vi "RemoteVI Menu Click.vi"(0 "hWnd":u64, 1 "button down?":bool, 5 "menus":T1(array[cluster]), 7 "k":i32, 9 "point":cluster{"x":i32, "y":i32}, 11 "error in":errorcluster) -> (4 "handled?":bool, 15 "error out":errorcluster)   [LabVIEW 2020, in "RemoteVI.lvlib"]
doc: "A remote click on an open LabVIEW menu window menus[k] (RemoteVI List Menus.vi, deepest first), done with keys only - no cursor and no window is moved, so every menu stays where LabVIEW put it. A BUTTON-DOWN: on a parent menu (k > 0) on the item that opened the open submenu nothing happens (as locally); otherwise the k submenus above are closed with VK_LEFT (RemoteVI Close Submenus.vi), the highlight is moved onto the clicked item (RemoteVI Highlight Menu Row.vi, VK_DOWN / VK_UP) and, when the item is under the click, VK_RETURN is posted - it chooses the item, or opens its submenu next to the menu when it has one (measured on LabVIEW 2025: plot legend, ring and shortcut menus). A click on a separator or a disabled item moves the highlight but chooses nothing. The menu pointer state (RemoteVI Menu Pointer.vi) records the click as navigated and dwelled (no hover action follows) and sets swallow up, so the matching button-up is not posted. A BUTTON-UP on a menu is dropped (the menu was already handled on the down; the release of the click that opened a menu must not choose an item). handled? is FALSE - the caller then clicks with the mouse path - when the window takes no keys: it showed no highlight even after a VK_DOWN probe (colour picker, line width popup; recorded as state.plain, and a button-up on it is passed on too), or when such a popup is open above the clicked parent (it takes no VK_LEFT, measured). No VI Server call."
uses:
  RemoteVI.lvlib
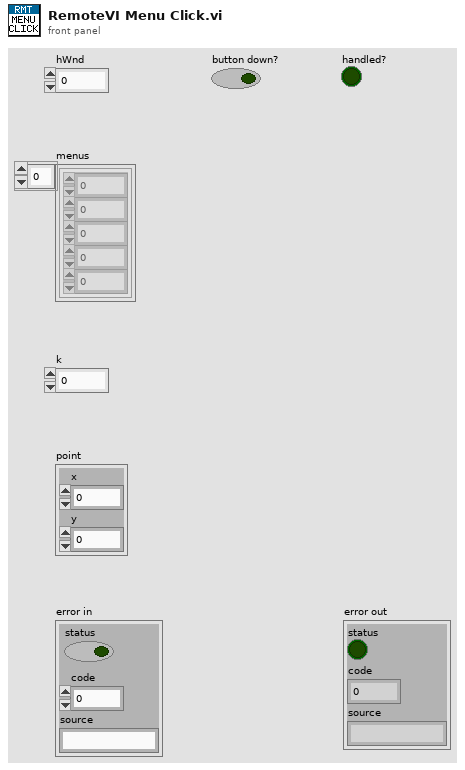
[diagram p1: front panel]
types:
  T1 = cluster{"hwnd":u64, "x":i32, "y":i32, "w":i32, "h":i32}[]
  T2 = cluster{"hwnd":u64, "x":i32, "y":i32, "w":i32, "h":i32}
  T3 = cluster{"active":bool, "x":i32, "y":i32, "moved":u32, "navigated":bool, "menu":u64, "top":i32, "hit":bool, "row since":u32, "dwelled":bool, "plain":u64, "swallow up":bool}
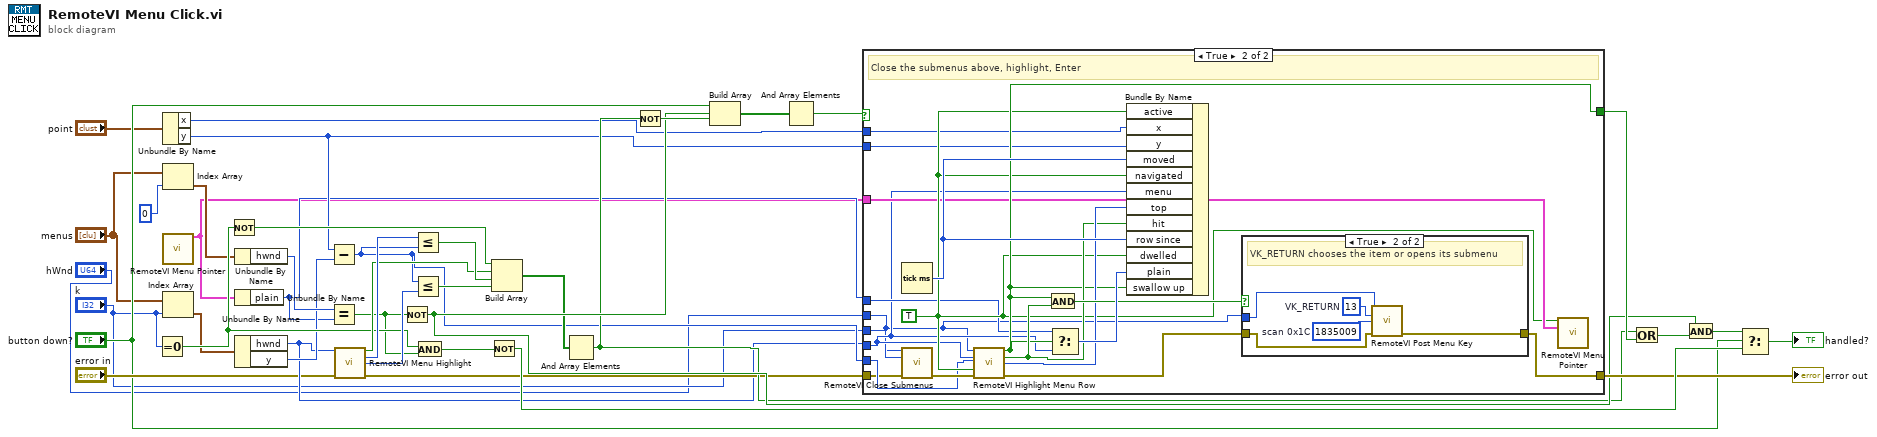
[diagram p0: block diagram]
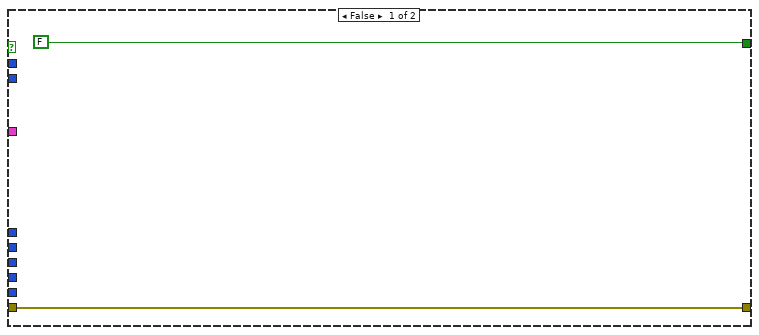
[diagram p2: hidden frame]
diagram:
  n1 = Equal To 0?(x="k") -> (x = 0?=w18:bool)
  n2 = Unbundle By Name("point") -> ("x"=w9:i32, "y"=w10:i32)
  n3 = Index Array(array="menus", index=0) -> (element=w15:T2)
  n4 = call "RemoteVI Menu Pointer.vi"() -> ("state"=w7:T3)  [unwired: 15 in]
  n5 = Index Array(array="menus", index="k") -> (element=w11:T2)
  n6 = Not(x=w18) -> (.not. x?=w19:bool)
  n7 = Unbundle By Name(w15) -> ("hwnd"=w16:u64)
  n8 = Unbundle By Name(w7) -> ("plain"=w8:u64)
  n9 = Unbundle By Name(w11) -> ("hwnd"=w12:u64, "y"=w13:i32)
  n10 = Subtract(x=w10, y=w13) -> (x-y=w20:i32)
  n11 = Equal?(x=w16, y=w8) -> (x = y?=w17:bool)
  n12 = call "RemoteVI Menu Highlight.vi"("hwnd"=w12, "error in"="error in") -> ("found?"=w21:bool, "top"=w22:i32, "bottom"=w23:i32, "error out"=w24:errorcluster)  [unwired: 7 in, 3 out]
  n13 = Not(x=w17) -> (.not. x?=w29:bool)
  n14 = Less Or Equal?(x=w22, y=w20) -> (x <= y?=w25:bool)
  n15 = Less Or Equal?(x=w20, y=w23) -> (x <= y?=w26:bool)
  n16 = And(x=w18, y=w17) -> (x .and. y?=w37:bool)
  n17 = Not(x=w37) -> (.not. x?=w38:bool)
  n18 = Build Array(w19, w21, w25, w26) -> (w27:bool[])
  n19 = And Array Elements(Boolean array=w27) -> (logical AND=w28:bool)
  n20 = Not(x=w28) -> (.not. x?=w30:bool)
  n21 = Build Array("button down?", w29, w30) -> (w31:bool[])
  n22 = And Array Elements(Boolean array=w31) -> (logical AND=w32:bool)
  n23 = case shown="True" w32 {
    tunnel: "hWnd" -> [_ w43]
    tunnel: "k" -> [_ w44]
    tunnel: w7 -> [_ w47]
    tunnel: w9 -> [_ w48]
    tunnel: w10 -> [_ w49]
    tunnel: w12 -> [_ w45]
    tunnel: w8 -> [_ w50]
    tunnel: w24 -> [w40 w42]
    tunnel: w20 -> [_ w46]
    tunnel: [FALSE w53] -> w34
    tunnel: [w40 w58] -> w33
    frame False {
    }
    frame True {
      w52 = TRUE
      # "Close the submenus above, highlight, Enter"
      n24 = Tick Count (ms)() -> (millisecond timer value=w59:u32)
      n25 = call "RemoteVI Close Submenus.vi"("hWnd"=w43, "count"=w44, "error in"=w42) -> ("error out"=w51:errorcluster)  [unwired: 12 in]
      n26 = call "RemoteVI Highlight Menu Row.vi"("hWnd"=w43, "menu"=w45, "y"=w46, "probe?"=w52, "error in"=w51) -> ("keyed?"=w53:bool, "hit?"=w54:bool, "top"=w55:i32, "error out"=w56:errorcluster)  [unwired: 6 in, 1 out]
      n27 = And(x=w53, y=w54) -> (x .and. y?=w57:bool)
      n28 = Select(t=w50, s=w53, f=w45) -> (s? t:f=w60:u64)
      n29 = Bundle By Name(cluster=w47, "active"=w52, "x"=w48, "y"=w49, "moved"=w59, "navigated"=w52, "menu"=w45, "top"=w55, "hit"=w54, "row since"=w59, "dwelled"=w52, "plain"=w60, "swallow up"=w53) -> (w61:T3)
      n30 = case shown="True" w57 {
        tunnel: w43 -> [_ w64]
        tunnel: w56 -> [w62 w63]
        tunnel: [w62 w67] -> w58
        frame False {
        }
        frame True {
          w66 = i64 1835009  # scan 0x1C
          w65 = u64 13  # VK_RETURN
          # "VK_RETURN chooses the item or opens its submenu"
          n31 = call "RemoteVI Post Menu Key.vi"("hWnd"=w64, "vk"=w65, "key lParam"=w66, "error in"=w63) -> ("error out"=w67:errorcluster)  [unwired: 11 in]
        }
      }
      n32 = call "RemoteVI Menu Pointer.vi"("write?"=w52, "state in"=w61) -> ()  [unwired: 13 in, 1 out]
    }
  }
  "error out" <- w33
  n33 = Or(x=w28, y=w34) -> (x .or. y?=w35:bool)
  n34 = And(x=w29, y=w35) -> (x .and. y?=w36:bool)
  n35 = Select(t=w36, s="button down?", f=w38) -> (s? t:f=→"handled?":bool)
